vi "DumpFileLoop.vi"(11 "DumpFileQueue":T1) -> ()   [LabVIEW 2025]
uses:
  DumpFileQueue.ctl
  DumpFileEvent.ctl
  DumpFileAction.ctl
  DumpFileState.ctl
  Communication/global_stop.vi
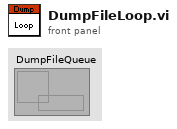
[diagram p1: front panel]
types:
  T1 = typedef "DumpFileQueue.ctl" = refnum<queue>
  T2 = typedef "DumpFileState.ctl" = cluster{"Path":path, "refnum":refnum<file>, "Lines":i32}
  T3 = typedef "DumpFileAction.ctl" = enum16{"StartNew", "StartAppend", "Data", "Close"}
  T4 = typedef "DumpFileEvent.ctl" = cluster{"Path":path, "DumpFileAction":T3, "Data":dbl[][]}
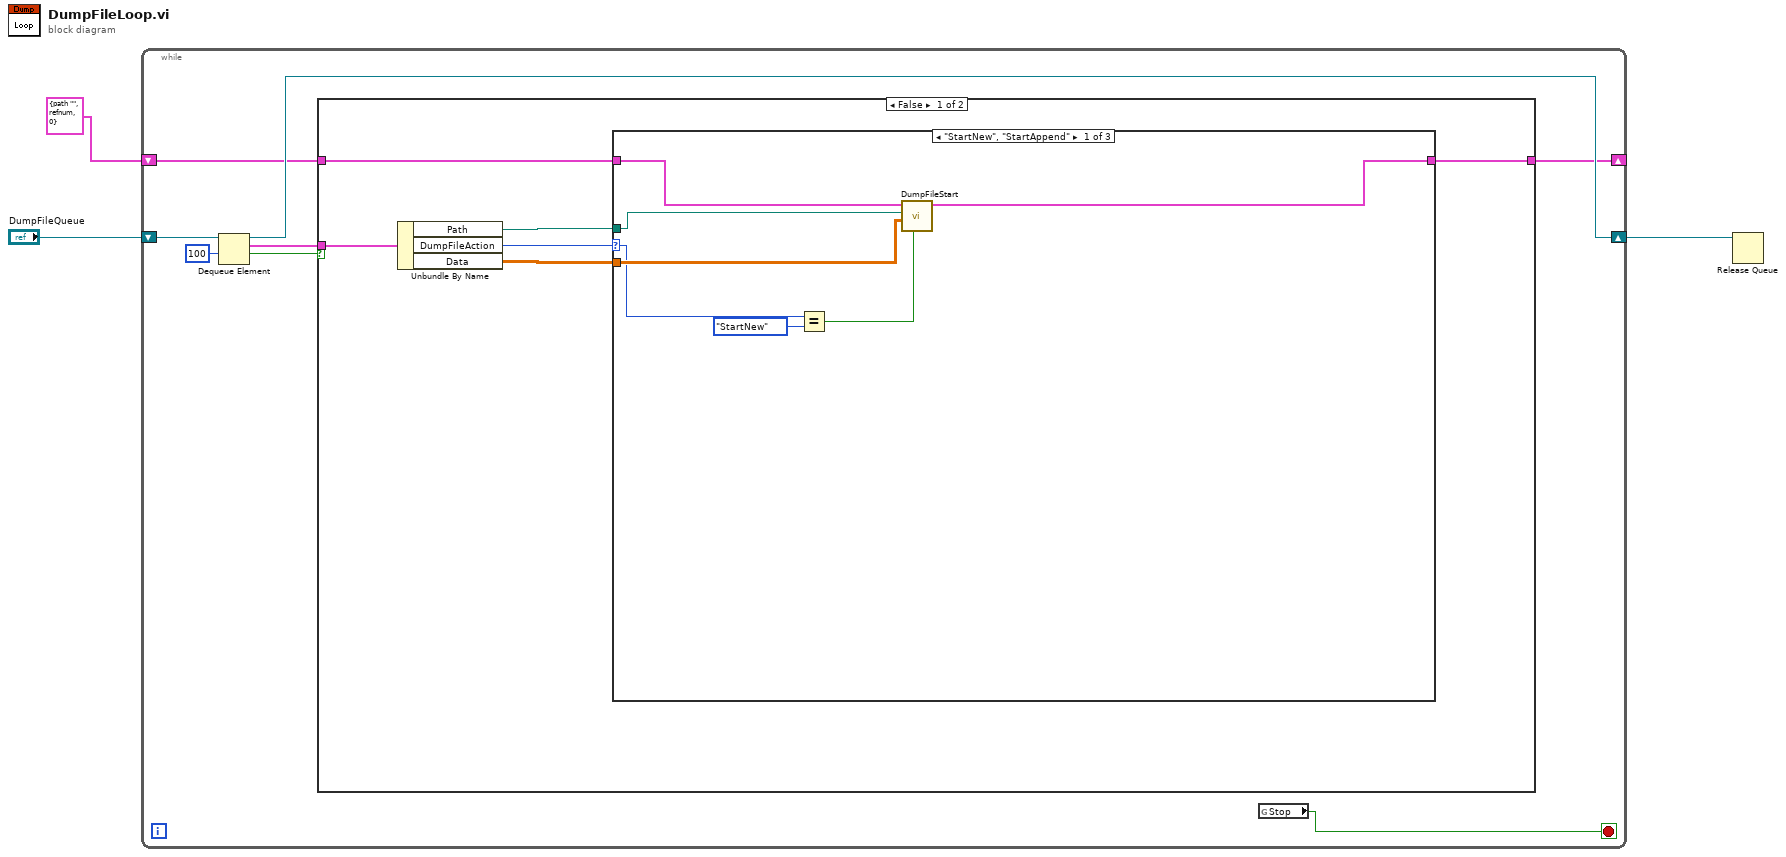
[diagram p0: block diagram]
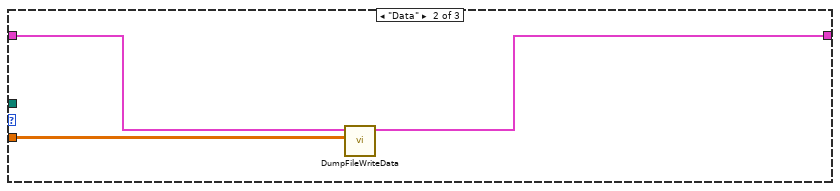
[diagram p2: hidden frame]
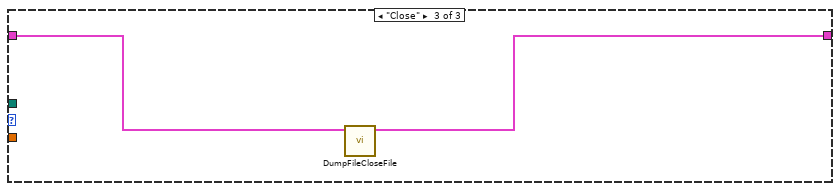
[diagram p3: hidden frame]
diagram:
  n1 = while {
    shift-right: [w7] -> w1
    shift-left: "DumpFileQueue" -> [w11]
    shift-right: [w5] -> _
    shift-left: T2 {"Path"=path "", "refnum"=refnum, "Lines"=0} ("DumpFileState") -> [w6]
    stop <- w4 stop-if-true
    n2 = Dequeue Element(queue=w11, timeout in ms (-1)=100) -> (queue out=w7:T1, element=w8:T4, timed out?=w9:bool)  [unwired: 1 in, 1 out]
    n3 = case shown="False" w9 {
      tunnel: w8 -> [w17 _]
      tunnel: w6 -> [w16 w30]
      tunnel: [w15 w30] -> w5
      frame False {
        n4 = Unbundle By Name(w17) -> ("Path"=w13:path, "DumpFileAction"=w14:T3, "Data"=w12:dbl[][])
        n5 = case shown="\"StartNew\", \"StartAppend\"" w14 {
          selector: w14 -> [w20 _ _]
          tunnel: w16 -> [w24 w26 w28]
          tunnel: [w23 w27 w29] -> w15
          tunnel: w13 -> [w22 _ _]
          tunnel: w12 -> [w21 w25 _]
          frame "StartNew", "StartAppend" {
            n6 = Equal?(x=w20, y=DumpFileAction."StartNew") -> (x = y?=w18:bool)
            n7 = call "DumpFileStart.vi"("Overwrite"=w18, "Data"=w21, "Path"=w22, "DumpFileState"=w24) -> ("DumpFileState out"=w23:T2)  [unwired: 7 in]
          }
          frame "Data" {
            n8 = call "DumpFileWriteData.vi"("Data"=w25, "DumpFileState"=w26) -> ("DumpFileState out"=w27:T2)  [unwired: 9 in]
          }
          frame "Close" {
            n9 = call "DumpFileCloseFile.vi"("DumpFileState"=w28) -> ("DumpFileState out"=w29:T2)  [unwired: 10 in]
          }
        }
      }
      frame True {
      }
    }
    n10 = global read "global_stop.vi" "Stop"() -> (w4:bool)
  }
  n11 = Release Queue(queue=w1) -> ()  [unwired: 2 in, 3 out]
